vi "VIH Utility - FILE - Validate File or Directory Path.vi"(8 "error in":errorcluster, 11 "Path":path) -> (0 "error out":errorcluster, 1 "directory":bool, 2 "file":bool, 3 "dup Path":path, 4 "size":i32)   [LabVIEW 2014]
doc: "::: VI Helpeks :::\nCopyright (c) 2000-2026 Konstantin Shifershteyn. All rights reserved."
panel:
  # "VI Helpeks\nCopyright (c) 2012-2026 Konstantin Shifershteyn"
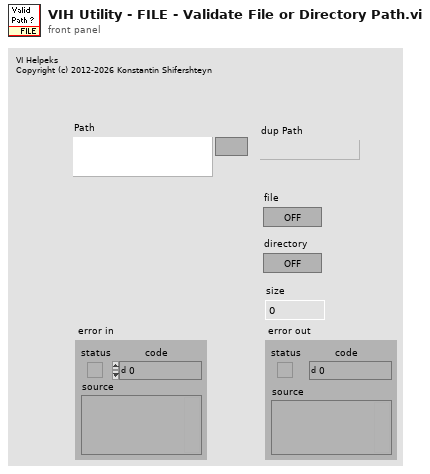
[diagram p1: front panel]
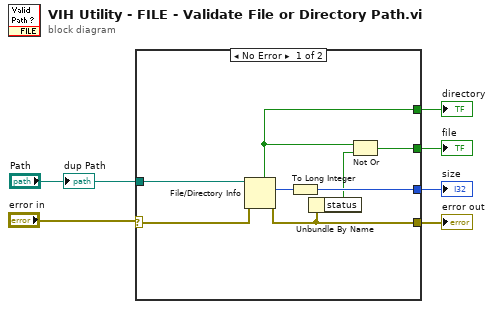
[diagram p0: block diagram]
diagram:
  n1 = case shown="No Error" "error in" {
    selector: "error in" -> [w8 w15]
    tunnel: "Path" -> [w10 _]
    tunnel: [w13 _] -> w4
    tunnel: [w14 w15] -> w3
    tunnel: [w12 _] -> w2
    tunnel: [w11 _] -> w1
    frame No Error {
      n2 = File/Directory Info(path=w10, error in=w8) -> (directory=w13:bool, size=w7:i64, error out=w14:errorcluster)  [unwired: 4 out]
      n3 = To Long Integer(number=w7) -> (32bit integer=w11:i32)
      n4 = Unbundle By Name(w14) -> ("status"=w9:bool)
      n5 = Not Or(1:w9, 2:w13) -> (0:w12:bool)
    }
    frame Error {
    }
  }
  "file" <- w2
  "directory" <- w4
  "error out" <- w3
  "size" <- w1
  "dup Path" <- "Path"
